vi "Set Antenna Pol.vi"(8 "error in (no error)":errorcluster, 11 "CO3000 in":refnum<class "CO3000.lvclass">) -> (0 "error out":errorcluster, 3 "CO3000 out":refnum<class "CO3000.lvclass">)   [LabVIEW 2023, in "Turn Table and Mast.lvlib" / "CO3000.lvclass"]
uses:
  CO3000.lvclass
  CO3000.lvclass/CO3000.ctl
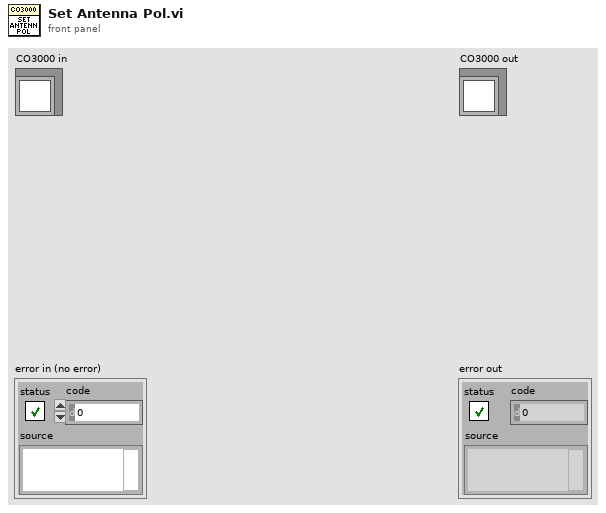
[diagram p1: front panel]
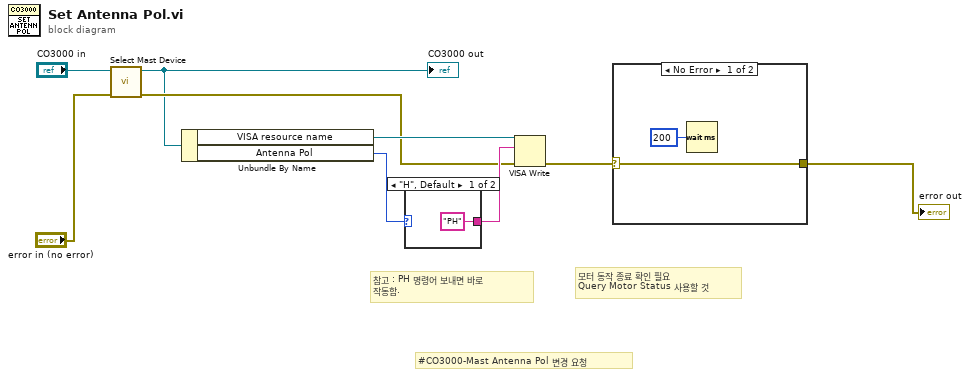
[diagram p0: block diagram]
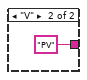
[diagram p3: hidden frame]
diagram:
  # "#CO3000-Mast Antenna Pol 변경 요청"
  # "모터 동작 종료 확인 필요\nQuery Motor Status 사용할 것"
  # "참고 : PH 명령어 보내면 바로\n작동함."
  n1 = call "Select Mast Device.vi"("error in (no error)"="error in (no error)", "CO3000 in"="CO3000 in") -> ("error out"=w4:errorcluster, "CO3000 out"=w3:refnum<class "CO3000.lvclass">)  [unwired: 8 in]
  "CO3000 out" <- w3
  n2 = Unbundle By Name(w3) -> ("VISA resource name"=w7:refnum<visa-resource-name>, "Antenna Pol"=w8:enum16{"H", "V"})
  n3 = case shown="\"H\", Default" w8 {
    tunnel: ["PH" ("버퍼 쓰기") "PV" ("버퍼 쓰기")] -> w9
    frame "H", Default {
    }
    frame "V" {
    }
  }
  n4 = VISA Write(VISA resource name=w7, write buffer=w9, error in (no error)=w4) -> (error out=w2:errorcluster)  [unwired: 2 out]
  n5 = case shown="No Error" w2 {
    selector: w2 -> [w12 w14]
    tunnel: [w12 w14] -> w1
    frame No Error {
      n6 = Wait (ms)(milliseconds to wait=u32 200) -> ()  [unwired: 1 out]
    }
    frame Error {
    }
  }
  "error out" <- w1
